vi "Linker.Find Tests and Suites.vi"(11 "Linker:Read Info From File":T2(array[cluster])) -> (1 "All VIs defining a Test Runner":path[](array[path]), 2 "All VIs defining a suite":path[](array[path]), 3 "All VIs defining a test (excluding those defining a suite)":path[](array[path]))   [LabVIEW 2020, in "Caraya.lvlib" / "Test Runner.lvclass"]
uses:
  Test Runner.lvclass
  <vilib>/Utility/lvfile.llb/LVFileType.ctl
  Caraya.lvlib
  <vilib>/Utility/lvfile.llb/NI_FileType.lvlib
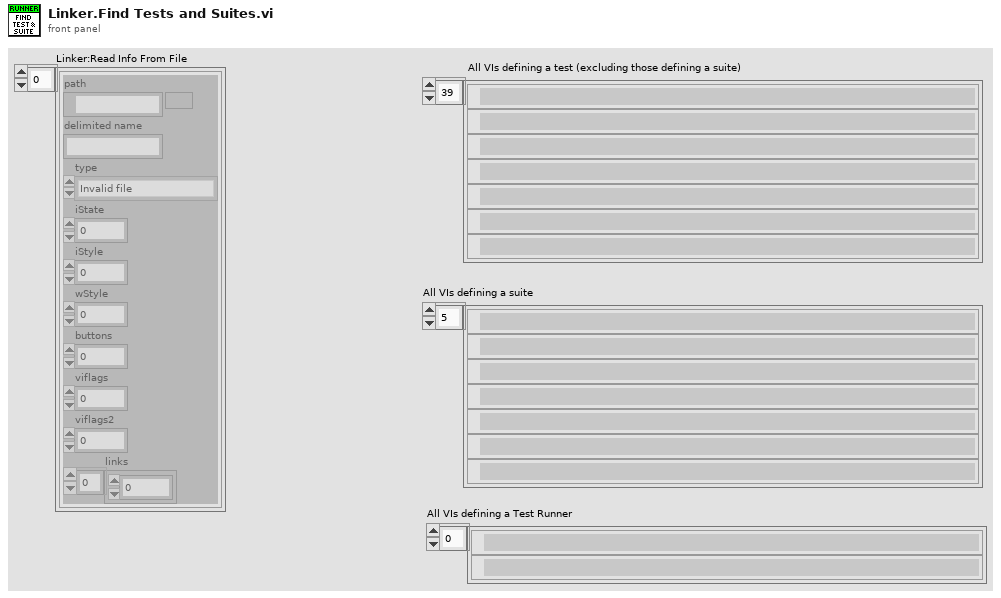
[diagram p1: front panel]
types:
  T1 = typedef "NI_FileType.lvlib/LVFileType.ctl" = enum32{"Invalid file", "Unknown type", "Instrument", "Control", "Polymorphic VI", "Project", "Library", "LVClass", "XControl", "XNode", "Shared library", ".NET assembly", "ActiveX interface", "CIN", "Run-time menu", "Palette menu", "Help file", "LLB", "XNode Edit Dependency", "Class Private Data Control", "Statechart", "MathScript .m file", "Ladder Diagram", "LVLibp", "XNode Build Dependency"}
  T2 = cluster{"path":path, "delimited name":string, "type":T1, "iState":u32, "iStyle":u16, "wStyle":u16, "buttons":u16, "viflags":u32, "viflags2":u32, "links":u32[]}[]
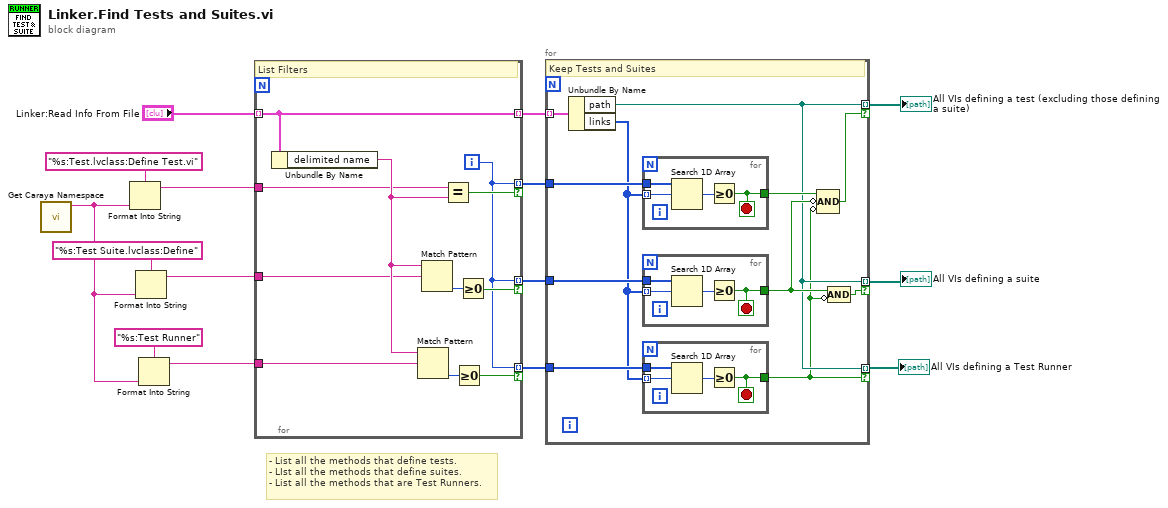
[diagram p0: block diagram]
diagram:
  # "- List all the methods that define tests.\n- LIst all the methods that define suites.\n- List all the methods that are Test Runners."
  n1 = call "Get Caraya Namespace.vi"() -> ("Namespace"=w2:string)  [unwired: 10 in, 1 out]
  n2 = Format Into String(format string="%s:Test.lvclass:Define Test.vi" ("pattern"), w2) -> (resulting string=w6:string)  [unwired: 2 in, 1 out]
  n3 = Format Into String(format string="%s:Test Suite.lvclass:Define" ("pattern"), w2) -> (resulting string=w4:string)  [unwired: 2 in, 1 out]
  n4 = Format Into String(format string="%s:Test Runner" ("pattern"), w2) -> (resulting string=w1:string)  [unwired: 2 in, 1 out]
  n5 = for {
    tunnel: "Linker:Read Info From File" -> [w23] mode=indexing
    tunnel: [w20] -> w15 mode=indexing if=w25
    tunnel: [w20] -> w14 mode=indexing if=w24
    tunnel: [w23] -> w13 mode=indexing
    tunnel: [w20] -> w9 mode=indexing if=w19
    tunnel: w6 -> [w18]
    tunnel: w4 -> [w17]
    tunnel: w1 -> [w16]
    i -> [w20]
    # "List Filters"
    n6 = Unbundle By Name(w23) -> ("delimited name"=w21:string)
    n7 = Match Pattern(string=w21, regular expression=w16) -> (offset past match=w22:i32)  [unwired: 1 in, 3 out]
    n8 = Match Pattern(string=w21, regular expression=w17) -> (offset past match=w26:i32)  [unwired: 1 in, 3 out]
    n9 = Equal?(x=w18, y=w21) -> (x = y?=w25:bool)
    n10 = Greater Or Equal To 0?(x=w22) -> (x >= 0?=w19:bool)
    n11 = Greater Or Equal To 0?(x=w26) -> (x >= 0?=w24:bool)
  }
  n12 = for {
    tunnel: w13 -> [w33] mode=indexing
    tunnel: w15 -> [w37]
    tunnel: [w28] -> w11 mode=indexing if=w34
    tunnel: w14 -> [w36]
    tunnel: [w28] -> w10 mode=indexing if=w30
    tunnel: w9 -> [w32]
    tunnel: [w28] -> w8 mode=indexing if=w27
    # "Keep Tests and Suites"
    n13 = Unbundle By Name(w33) -> ("path"=w28:path, "links"=w31:u32[])
    n14 = for {
      tunnel: w37 -> [w49]
      tunnel: w31 -> [w48] mode=indexing
      tunnel: [w46] -> w35
      stop <- w46 stop-if-true
      n15 = Search 1D Array(1D array=w49, element=w48) -> (index of element=w47:i32)  [unwired: 1 in]
      n16 = Greater Or Equal To 0?(x=w47) -> (x >= 0?=w46:bool)
    }
    n17 = for {
      tunnel: w36 -> [w45]
      tunnel: w31 -> [w44] mode=indexing
      tunnel: [w42] -> w29
      stop <- w42 stop-if-true
      n18 = Search 1D Array(1D array=w45, element=w44) -> (index of element=w43:i32)  [unwired: 1 in]
      n19 = Greater Or Equal To 0?(x=w43) -> (x >= 0?=w42:bool)
    }
    n20 = for {
      tunnel: w32 -> [w41]
      tunnel: w31 -> [w40] mode=indexing
      tunnel: [w38] -> w27
      stop <- w38 stop-if-true
      n21 = Search 1D Array(1D array=w41, element=w40) -> (index of element=w39:i32)  [unwired: 1 in]
      n22 = Greater Or Equal To 0?(x=w39) -> (x >= 0?=w38:bool)
    }
    n23 = Compound Arithmetic op=AND(w35, invert w29, invert w27) -> (w34:bool)
    n24 = Compound Arithmetic op=AND(w29, invert w27) -> (w30:bool)
  }
  "All VIs defining a test (excluding those defining a suite)" <- w11
  "All VIs defining a suite" <- w10
  "All VIs defining a Test Runner" <- w8
